vi "Save Entry.vi"(7 "Time Entry Store in":refnum<class "Time Entry Store.lvclass">, 8 "error in (no error)":errorcluster, 10 "Project Store":refnum<class "Project Store.lvclass">, 11 "Time Entry":T1) -> (0 "error out":errorcluster, 5 "Time Entry Store out":refnum<class "Time Entry Store.lvclass">)   [LabVIEW 2024, in "Time Entry Store.lvclass"]
doc: "Saves a time entry: creates its row, or overwrites the row with the same ID. Project Store is optional and only used to write the Project Name and Task Name labels. The parent class has no storage: it returns empty results and does nothing. Time Entry Store-INI overrides it.\n\nGenerated by: Claude"
uses:
  Time Entry Store.lvclass
  Project Store/Project Store.lvclass
  Rows/Time Entry.ctl
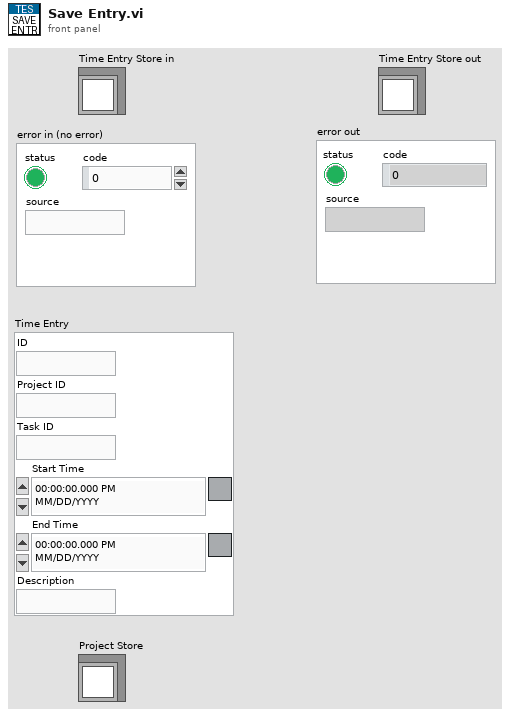
[diagram p1: front panel]
types:
  T1 = typedef "Time Entry.ctl" = cluster{"ID":string, "Project ID":string, "Task ID":string, "Start Time":timestamp, "End Time":timestamp, "Description":string}
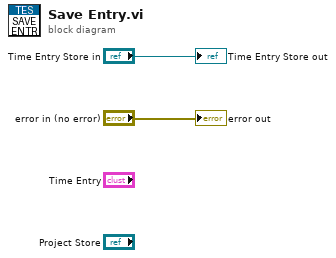
[diagram p0: block diagram]
diagram:
  "Time Entry Store out" <- "Time Entry Store in"
  "error out" <- "error in (no error)"
